vi "Number Search.vi"(10 "Target Value":i32, 11 "Upper Limit":i32) -> (3 "Output":i32[](array[numeric]))   [LabVIEW 2026]
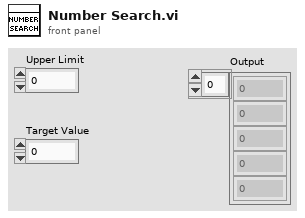
[diagram p1: front panel]
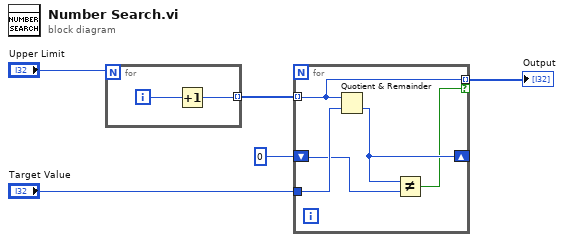
[diagram p0: block diagram]
diagram:
  n1 = for {
    N: "Upper Limit" -> [_]
    tunnel: [w6] -> w4 mode=indexing
    i -> [w7]
    n2 = Increment(x=w7) -> (x+1=w6:i32)
  }
  n3 = for {
    tunnel: w4 -> [w9] mode=indexing
    tunnel: "Target Value" -> [w12]
    shift-right: [w10] -> _
    shift-left: 0 -> [w11]
    tunnel: [w9] -> w1 mode=indexing if=w8
    n4 = Quotient & Remainder(x=w9, y=w12) -> (floor(x/y)=w10:i32)  [unwired: 1 out]
    n5 = Not Equal?(x=w10, y=w11) -> (x != y?=w8:bool)
  }
  "Output" <- w1
